vi "GetRightClickMenu.vi"(0 "reference":refnum<class "StateDiagramGraph.lvclass">, 5 "error in (no error)":errorcluster) -> (14 "reference out":refnum<class "StateDiagramGraph.lvclass">, 15 "Array":string[](array[string]), 16 "Found":bool, 19 "error out":errorcluster)   [LabVIEW 2020, in "StateDiagramGraph.lvclass"]
doc: "GetRightClickMenu"
uses:
  <resource>/Framework/Providers/Open_GDS/UML/StateDiagramGraph_class/StateDiagramGraph.lvclass
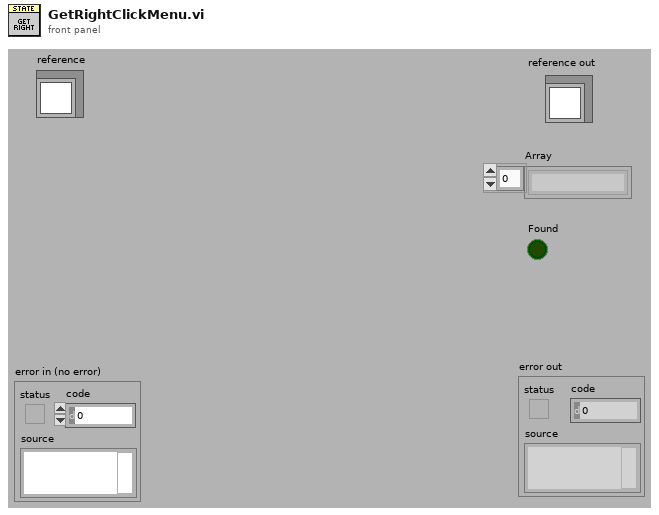
[diagram p1: front panel]
types:
  T1 = typedef "StateDiagramGraph.lvclass/ObjectAttributes.ctl" = cluster{"StateDiagramData":T2}
  T2 = typedef "StateDiagramGraph.lvclass/StateDiagramData.ctl" = cluster{"VI-Path":path, "ShowOption":T3}
  T3 = typedef "StateDiagramGraph.lvclass/ViPathShowOption.ctl" = enum16{"Don't Show", "Show Relative Path", "Show Absolute Path"}
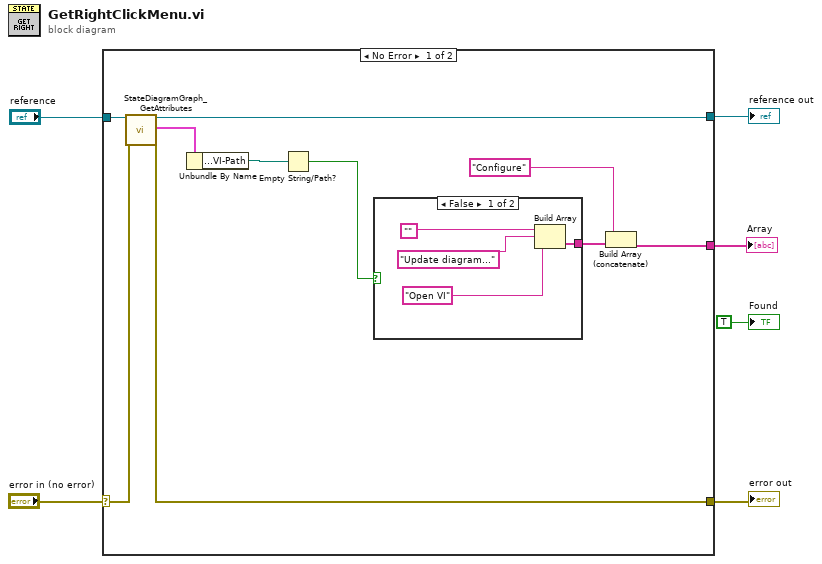
[diagram p0: block diagram]
diagram:
  n1 = case shown="No Error" "error in (no error)" {
    selector: "error in (no error)" -> [w16 w21]
    tunnel: "reference" -> [w15 w22]
    tunnel: [w13 w21] -> w4
    tunnel: [w14 w22] -> w3
    tunnel: [w11 _] -> w2
    frame No Error {
      n2 = call <resource>:"StateDiagramGraph_GetAttributes.vi"("reference in"=w15, "error in (no error)"=w16) -> ("reference out"=w14:refnum<class "StateDiagramGraph.lvclass">, "Data"=w7:T1, "error out"=w13:errorcluster)  [unwired: 1 in, 14 out]
      n3 = Unbundle By Name(w7) -> ("StateDiagramData.VI-Path"=w12:path)
      n4 = Empty String/Path?(string/path=w12) -> (empty?=w10:bool)
      n5 = case shown="False" w10 {
        tunnel: [w18 _] -> w8
        frame False {
          n6 = Build Array("", "Update diagram...", "Open VI") -> (w18:string[])
        }
        frame True {
        }
      }
      n7 = Build Array (concatenate)("Configure", w8) -> (w11:string[])
    }
    frame Error {
    }
  }
  "reference out" <- w3
  "error out" <- w4
  "Array" <- w2
  "Found" <- TRUE ("Found")
